vi "Create Blackboard.vi"(8 "error in (no error)":errorcluster, 10 "Max Readers":u32=64, 11 "Blackboard name":string="my_blackboard") -> (0 "error out":errorcluster, 3 "Blackboard Reference":T1 {"refnum" format="%.0x"})   [LabVIEW 2021, in "Iceoryx.lvlib"]
uses:
  Iceoryx.lvlib
  Refnum/Typedef/BB Refnum.ctl
  <vilib>/CIF Foundation/CIF Utilities/File/SubVIs/File Not Found Error Core.vi
  SubVIs/Convert Error Core.vi
  <vilib>/CIF Foundation/CIF Utilities/File/File_CIF_U.lvlib
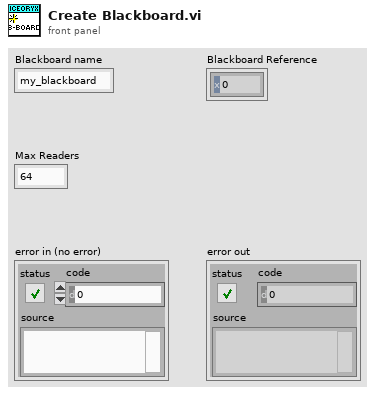
[diagram p1: front panel]
types:
  T1 = typedef "Iceoryx.lvlib/BB Refnum.ctl" = cluster{"refnum":u64, "BB":enum8{"bb"}}
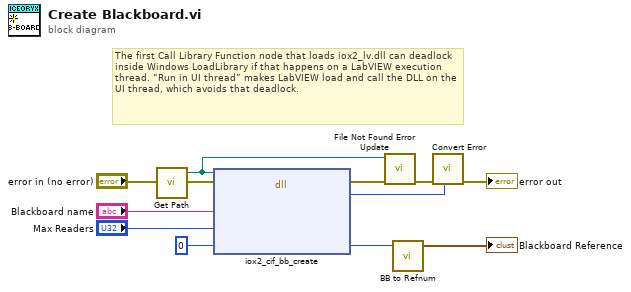
[diagram p0: block diagram]
diagram:
  # "The first Call Library Function node that loads iox2_lv.dll can deadlock inside Windows LoadLibrary if that happens on a LabVIEW execution thread. “Run in UI thread” makes LabVIEW load and call the DLL on the UI thread, which avoids that deadlock."
  n1 = call "Get Path.vi"() -> ("libiox2_cif path"=w2:path)  [unwired: 4 in]
  n2 = dll-call lib="D:/dev/iceoryx2_lvwrapper/dist/iox2_cif.dll" fn="iox2_cif_bb_create"(path in=w2, error in="error in (no error)", "name"="Blackboard name", "max_readers"="Max Readers", "bb"=u64 0) -> (error out=w6:errorcluster, "return type"=w3:i32, "bb"=w8:u64)  [unwired: 3 in, 1 out]
  n3 = call <vilib>:"File Not Found Error Update.vi"("error in"=w6, "path in"=w2) -> ("error out"=w5:errorcluster)  [unwired: 9 in]
  n4 = call "BB to Refnum.vi"("BB U64"=w8) -> ("BB Refnum"=→"Blackboard Reference":T1)  [unwired: 4 in]
  n5 = call "Convert Error.vi"("return type"=w3, "error in (no error)"=w5) -> ("error out"=→"error out":errorcluster)  [unwired: 9 in]
